vi "MB_ReadD.vi"(8 "error in":errorcluster, 11 "TCP Network Connection in":refnum<k5>) -> (0 "error out":errorcluster, 1 "Array":bool[](array[boolean]), 3 "TCP Network Connection out":refnum<k5>)   [LabVIEW 2018]
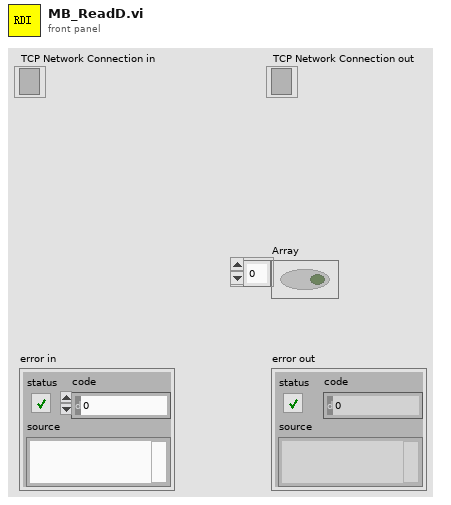
[diagram p1: front panel]
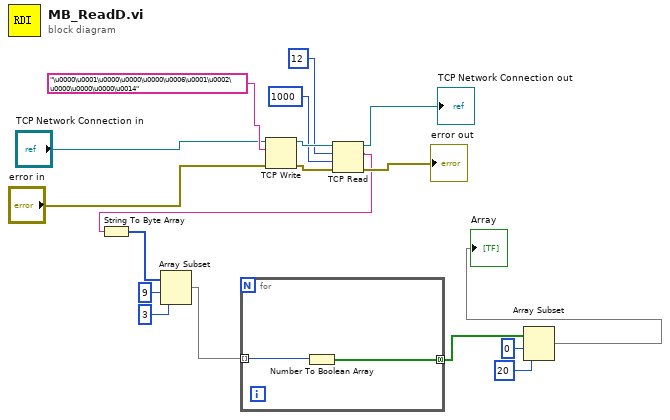
[diagram p0: block diagram]
diagram:
  n1 = TCP Write(connection ID="TCP Network Connection in", data in="\u0000\u0001\u0000\u0000\u0000\u0006\u0001\u0002\u0000\u0000\u0000\u0014", error in (no error)="error in") -> (connection ID out=w7:refnum<k5>, error out=w6:errorcluster)  [unwired: 1 in, 1 out]
  n2 = TCP Read(connection ID=w7, bytes to read=12, error in (no error)=w6, 9:1000 ("timeout ms (25000)")) -> (connection ID out=→"TCP Network Connection out":refnum<k5>, data out=w1:string, error out=→"error out":errorcluster)  [unwired: 1 in]
  n3 = String To Byte Array(string=w1) -> (unsigned byte array=w8:u8[])
  n4 = Array Subset(array=w8, index=9, length=3) -> (w11:u8[])
  n5 = for {
    tunnel: w11 -> [w20] mode=indexing
    tunnel: [w19] -> w14 mode=concatenating
    n6 = Number To Boolean Array(number=w20) -> (Boolean array=w19:bool[])
  }
  n7 = Array Subset(array=w14, index=0, length=20) -> (→"Array":bool[])
